vi "Bang Bang Temp Control.vi"(1 "Previous Heater State":bool, 2 "Temperature":dbl) -> (0 "New Heater State":bool)   [LabVIEW 2021]
uses:
  Temperature Limits.vi
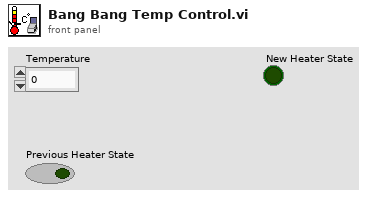
[diagram p1: front panel]
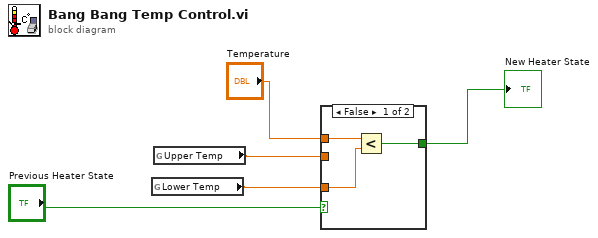
[diagram p0: block diagram]
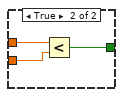
[diagram p2: hidden frame]
diagram:
  n1 = global read "Temperature Limits.vi" "Lower Temp"() -> (w1:dbl)
  n2 = global read "Temperature Limits.vi" "Upper Temp"() -> (w2:dbl)
  n3 = case shown="False" "Previous Heater State" {
    tunnel: "Temperature" -> [w8 w11]
    tunnel: w2 -> [_ w10]
    tunnel: [w7 w9] -> w4
    tunnel: w1 -> [w6 _]
    frame False {
      n4 = Less?(x=w8, y=w6) -> (x < y?=w7:bool)
    }
    frame True {
      n5 = Less?(x=w11, y=w10) -> (x < y?=w9:bool)
    }
  }
  "New Heater State" <- w4
